vi "Measurement Logic.vi"() -> ()   [LabVIEW 2022 SP3, in "Efficiency Sweep_Class D Amplifier.lvlib"]
uses:
  Efficiency Sweep_Class D Amplifier.lvlib
  Measurement Results.ctl
  <vilib>/Analysis/NI_AALBase.lvlib
  <instrlib>/niDCPower/nidcpower.llb/niDCPower Source Mode.ctl
  <instrlib>/niDCPower/nidcpower.llb/niDCPower Output Function.ctl
  <instrlib>/niDMM/nidmm.llb/niDMM Function.ctl
  <instrlib>/niDMM/nidmm.llb/niDMM Resolution in Digits.ctl
  <vilib>/Analysis/1siggen.llb/Ramp Pattern by Samples.vi
  <instrlib>/niDMM/nidmm.llb/niDMM Configure Measurement Digits.vi
  <vilib>/Plug-In SDKs/Measurements/Measure Call Context/Measure Call Context.lvclass
  Measurement Configuration.ctl
  shared/controls/weighting filter.ctl
  shared/controls/lowpass filter.ctl
  shared/controls/highpass filter.ctl
  shared/controls/units - snr.ctl
  shared/controls/audio controls.lvlib
  shared/controls/units - ratio.ctl
  shared/controls/digital output level units.ctl
  shared/controls/power measurement method.ctl
panel:
  out "XY Graph":cluster{"Array":dbl[], "Array":dbl[]}(graph)
  out "Spectrum":cluster{"x0":dbl, "dx":dbl, "magnitude":dbl[]}[](graph)
  out "Waveform Graph":waveform(dbl)[](graph)
  out "measure call context out":refnum<class "Measure Call Context.lvclass">
  in  "measure call context in":refnum<class "Measure Call Context.lvclass">
  out "measurement results":T1={"channel name"="0", "power supply voltage (V)"=[], "power supply current (A)"=[], "input power (W)"=[], "total output power (W)"=[], "power loss (W)"=[], "efficiency (%)"=[], "wfm - t0"=0.0, "wfm - dt"=1.9531249997269942e-05, "wfm - data"=array[12800 elements], "fft - f0"=0.0, "fft - df"=4.000000000559116, "fft - data"=array[6400 elements]}
  in  "measurement configuration":T2={"digital serial cfg file"="", "digital channel list"="7821\\PCMo 8", "master clock channel list"="7821\\PCMo 0", "output level start"=10.0, "output level stop"=60.0, "output sweep number of steps"=5, "output level units"=enum."% FS", "output range (pk-pk)"=15.0, "load impedance"=4.0, "signal phase"=0.0, "acq sampling rate"=51200.0, "min measurement cycles"=20, "min measurement time (s)"=0.1, "min settling cycles"=0, "min settling time (s)"=0.005, "acq channel"="PXI1Slot4/ai0", "band start"=20.0, "band stop"=20000.0, "weighting filter"=enum."Linear", "highpass filter"=enum."DC", "lowpass filter"=enum."No filter", "SNR units"=enum."dB", "THD+N units"=enum."dB", "THD units"=enum."dB", "gain units"=enum."dB", "power measurement method"=enum."DMM", "power measurement resource"="PXI1Slot9", "power supply voltage"=14.4, "power supply current limit"=1.2, "sense resistor (Ohms)"=0.01} {"band start" format="%0.2f"; "acq sampling rate" format="%0.2f"; "signal phase" format="%#_6p"}
  out "error out":errorcluster
  in  "error in":errorcluster
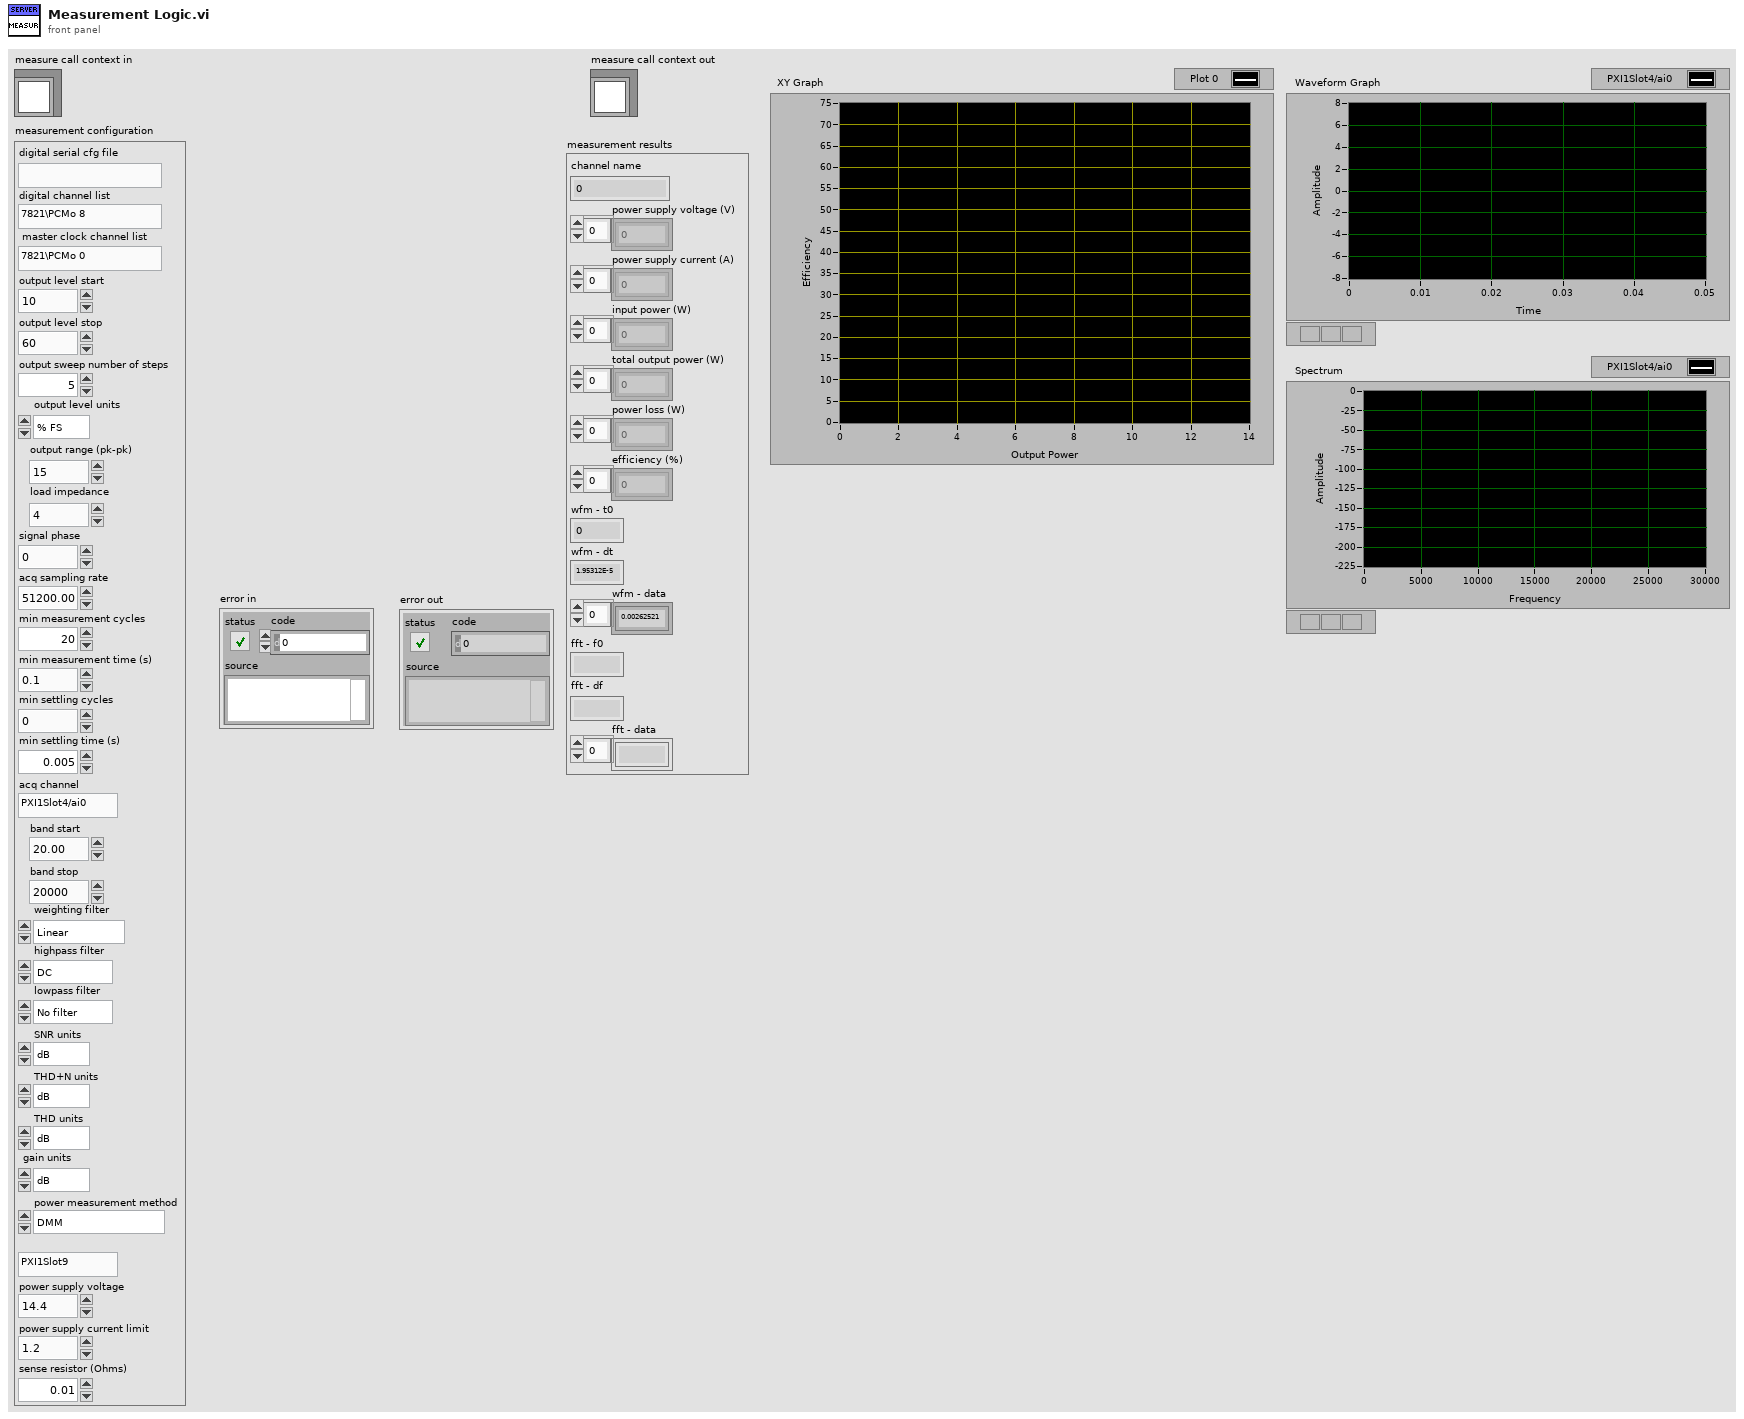
[diagram p1: front panel]
types:
  T1 = typedef "Efficiency Sweep_Class D Amplifier.lvlib/Measurement Results.ctl" = cluster{"channel name":string, "power supply voltage (V)":dbl[], "power supply current (A)":dbl[], "input power (W)":dbl[], "total output power (W)":dbl[], "power loss (W)":dbl[], "efficiency (%)":dbl[], "wfm - t0":dbl, "wfm - dt":dbl, "wfm - data":dbl[], "fft - f0":dbl, "fft - df":dbl, "fft - data":dbl[]}
  T2 = typedef "Efficiency Sweep_Class D Amplifier.lvlib/Measurement Configuration.ctl" = cluster{"digital serial cfg file":string, "digital channel list":string, "master clock channel list":string, "output level start":dbl, "output level stop":dbl, "output sweep number of steps":u32, "output level units":T3, "output range (pk-pk)":dbl, "load impedance":dbl, "signal phase":dbl, "acq sampling rate":dbl, "min measurement cycles":u32, "min measurement time (s)":dbl, "min settling cycles":u32, "min settling time (s)":dbl, "acq channel":string, "band start":dbl, "band stop":dbl, "weighting filter":T4, "highpass filter":T5, "lowpass filter":T6, "SNR units":T7, "THD+N units":T8, "THD units":T8, "gain units":T8, "power measurement method":T9, "power measurement resource":string, "power supply voltage":dbl, "power supply current limit":dbl, "sense resistor (Ohms)":dbl}
  T3 = typedef "audio controls.lvlib/digital output level units.ctl" = enum32{"% FS", "dBFS", "V"}
  T4 = typedef "weighting filter.ctl" = enum32{"Linear", "A-weighting", "B-weighting", "C-weighting"}
  T5 = typedef "highpass filter.ctl" = enum32{"DC", "AC"}
  T6 = typedef "lowpass filter.ctl" = enum32{"No filter", "AES17 20kHz", "AES17 40kHz"}
  T7 = typedef "audio controls.lvlib/units - snr.ctl" = enum32{"dB", "x/y"}
  T8 = typedef "audio controls.lvlib/units - ratio.ctl" = enum32{"dB", "%", "x/y"}
  T9 = typedef "power measurement method.ctl" = enum32{"SMU", "DMM"}
  T10 = typedef "niDMM Function.ctl" = enum16{"DC Volts", "AC Volts", "DC Current", "AC Current", "2-wire Resistance", "4-wire Resistance", "Diode", "Frequency", "Period", "AC Volts DC Coupled", "Capacitance", "Inductance", "Temperature"}
  T11 = typedef "niDCPower Output Function.ctl" = i32
  T12 = typedef "niDCPower Source Mode.ctl" = i32
  T13 = typedef "niDMM Resolution in Digits.ctl" = dbl
  T14 = typedef "single tone measurement settings (HW).ctl" = cluster{"digital channel list":string, "frame clock rate":dbl, "number of channels":u32, "channel length":u32, "bit depth":u32, "data justification":T15, "endianness":T16, "bit clock edge sync":T17, "frame sync edge for channel 0":T17, "channel 0 offset":u32, "master clock channel list":string, "master clock rate":dbl, "enable dither":bool, "logic level":T18, "signal frequency":dbl, "output level":dbl, "output level units":T3, "output range (pk-pk)":dbl, "load impedance":dbl, "signal phase":dbl, "acq sampling rate":dbl, "min measurement cycles":u32, "min measurement time (s)":dbl, "min settling cycles":u32, "min settling time (s)":dbl, "acq channel":string, "band start":dbl, "band stop":dbl, "weighting filter":T4, "highpass filter":T5, "lowpass filter":T6, "SNR units":T7, "THD+N units":T8, "THD units":T8, "gain units":T8}
  T15 = typedef "data justification.ctl" = enum32{"Left Justified", "Right Justified"}
  T16 = typedef "endianness.ctl" = enum32{"MSB First", "LSB First"}
  T17 = typedef "digital edge.ctl" = enum32{"Rising", "Falling"}
  T18 = typedef "logic level.ctl" = enum32{"3.3 V", "1.8 V", "1.2 V"}
  T19 = typedef "PCM tasks.ctl" = cluster{"PCM output task":T20, "PCM output task-clock":T20}
  T20 = typedef "PDM Acquisition Class Library.lvlib/PCM Output Task.lvclass/PCM Output Task DVR.ctl" = refnum<data-value>
  T21 = typedef "audio controls.lvlib/single tone audio measurements.ctl" = cluster{"channel":string, "frequency (Hz)":dbl, "amplitude (Vrms)":dbl, "amplitude (dBFS)":dbl, "phase (deg)":dbl, "SNR":dbl, "THD+N":dbl, "THD":dbl, "dynamic range (dB)":dbl, "gain":dbl, "SFDR (dBc)":dbl}
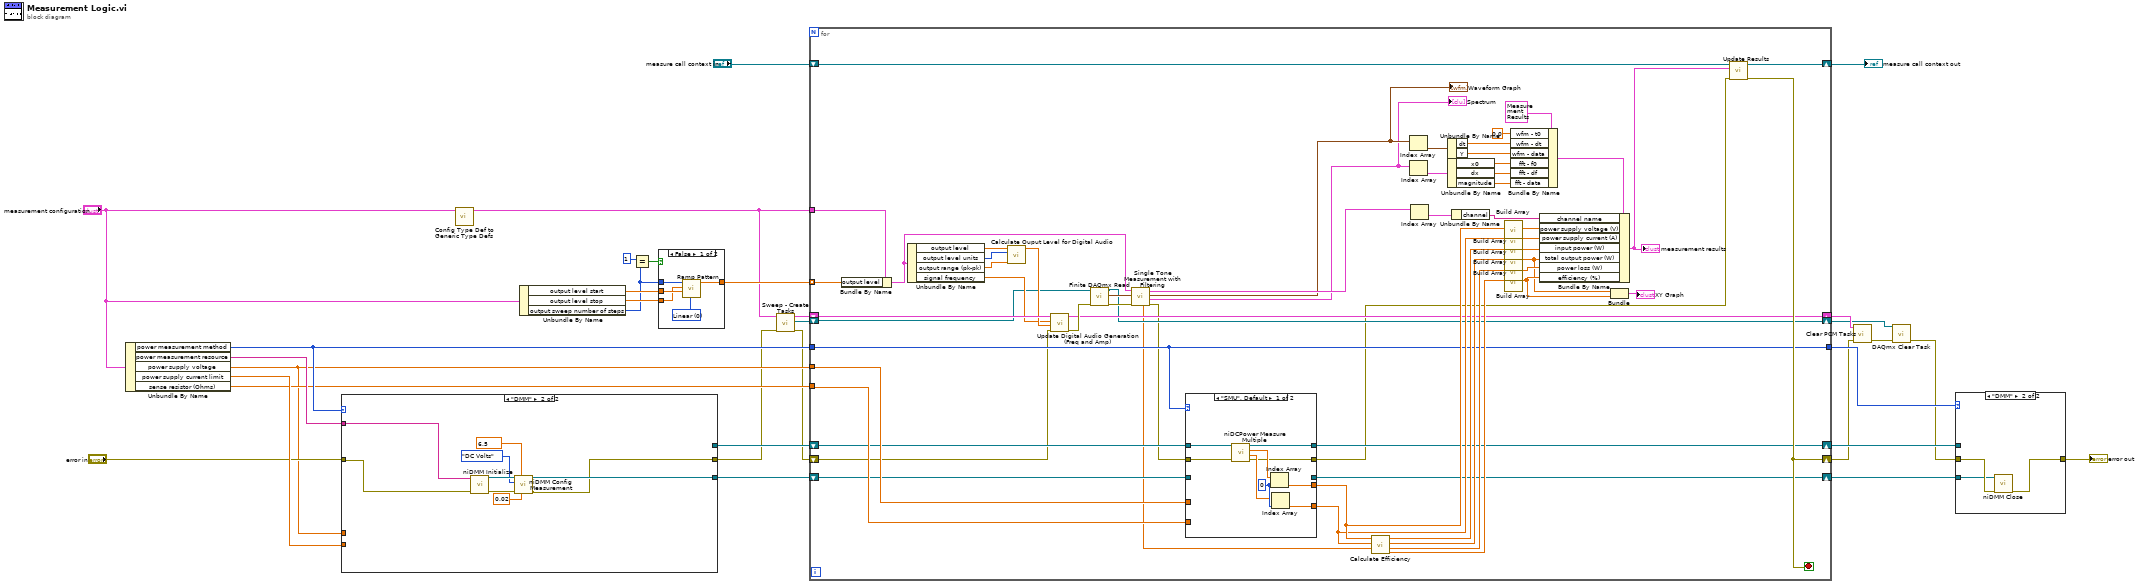
[diagram p0: block diagram]
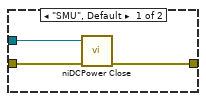
[diagram p2: hidden frame]
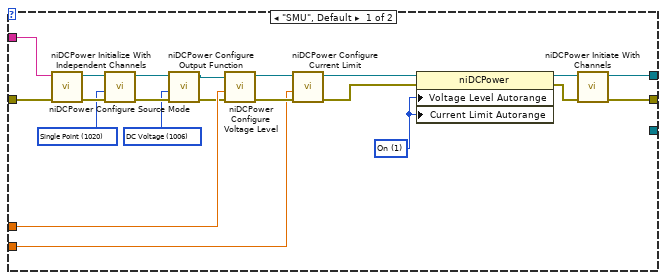
[diagram p3: hidden frame]
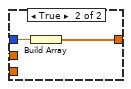
[diagram p4: hidden frame]
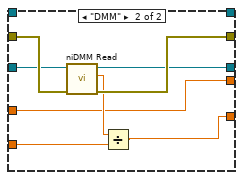
[diagram p5: hidden frame]
diagram:
  n1 = Unbundle By Name("measurement configuration") -> ("power measurement method"=w20:T9, "power measurement resource"=w23:string, "power supply voltage"=w18:dbl, "power supply current limit"=w22:dbl, "sense resistor (Ohms)"=w19:dbl)
  n2 = case shown="\"DMM\"" w20 {
    tunnel: w18 -> [w50 _]
    tunnel: w22 -> [w49 _]
    tunnel: [w35 _] -> w11
    tunnel: [w34 w57] -> w10
    tunnel: "error in" -> [w33 w61]
    tunnel: [_ w58] -> w12
    tunnel: w23 -> [w32 w53]
    frame "SMU", Default {
      w36 = 1 items=["Off", "On"] ("Source:DC Voltage:Current Limit Autorange")
      w37 = T11 1006 items=["DC Voltage"=1006, "DC Current"=1007, "Pulse Voltage"=1049, "Pulse Current"=1050] ("output function")
      w44 = T12 1020 items=["Single Point"=1020, "Sequence"=1021] ("source mode")
      n3 = call <instrlib>:"niDCPower Initialize With Independent Channels.vi"("error in (no error)"=w33, "resource name"=w32) -> ("error out"=w48:errorcluster, "instrument handle out"=w47:refnum<k15>)  [unwired: 8 in]
      n4 = call <instrlib>:"niDCPower Configure Source Mode.vi"("error in (no error)"=w48, "source mode"=w44, "instrument handle"=w47) -> ("error out"=w46:errorcluster, "instrument handle out"=w45:refnum<k15>)  [unwired: 7 out]
      n5 = call <instrlib>:"niDCPower Configure Output Function.vi"("error in (no error)"=w46, "output function"=w37, "instrument handle"=w45) -> ("error out"=w38:errorcluster, "instrument handle out"=w39:refnum<k15>)  [unwired: 1 in, 6 out]
      n6 = call <instrlib>:"niDCPower Configure Voltage Level.vi"("error in (no error)"=w38, "voltage level"=w50, "instrument handle"=w39) -> ("error out"=w51:errorcluster, "instrument handle out"=w52:refnum<k15>)  [unwired: 1 in, 6 out]
      n7 = call <instrlib>:"niDCPower Configure Current Limit.vi"("error in (no error)"=w51, "current limit"=w49, "instrument handle"=w52) -> ("error out"=w40:errorcluster, "instrument handle out"=w43:refnum<k15>)  [unwired: 2 in, 5 out]
      n8 = property class="niDCPower"(reference=w43, error in=w40, "Voltage Level Autorange"=w36, "Current Limit Autorange"=w36) -> (reference out=w42:refnum<k15>, error out=w41:errorcluster)
      n9 = call <instrlib>:"niDCPower Initiate With Channels.vi"("error in (no error)"=w41, "instrument handle"=w42) -> ("error out"=w34:errorcluster, "instrument handle out"=w35:refnum<k15>)  [unwired: 8 in]
    }
    frame "DMM" {
      w55 = T13 6.5 items=["3 1/2"=3.5, "4 1/2"=4.5, "5 1/2"=5.5, "6 1/2"=6.5, "7 1/2"=7.5] ("Resolution in Digits")
      n10 = call <instrlib>:"niDMM Initialize.vi"("error in (no error)"=w61, "Instrument Descriptor"=w53) -> ("error out"=w60:errorcluster, "instrument handle out"=w59:refnum<k15>)  [unwired: 8 in]
      n11 = call-poly <instrlib>:"niDMM Config Measurement.vi"("Range"=0.02, "Resolution in Digits"=w55, "error in (no error)"=w60, "Function"=niDMM_Function."DC Volts", "instrument handle"=w59) -> ("error out"=w57:errorcluster, "instrument handle out"=w58:refnum<k15>)  [unwired: 5 in]
    }
  }
  n12 = call "Config Type Def to Generic Type Defs.vi"("measurement configuration"="measurement configuration") -> ("single tone settings"=w9:T14)  [unwired: 9 in, 1 out]
  n13 = Unbundle By Name("measurement configuration") -> ("output level start"=w31:dbl, "output level stop"=w30:dbl, "output sweep number of steps"=w26:u32)
  n14 = Equal?(x=u32 1, y=w26) -> (x = y?=w27:bool)
  n15 = case shown="False" w27 {
    tunnel: w31 -> [w66 w68]
    tunnel: w30 -> [w65 _]
    tunnel: w26 -> [w64 _]
    tunnel: [w63 w67] -> w29
    frame False {
      w62 = u16 0 items=["Linear", "Logarithmic"] ("type")
      n16 = call-poly <vilib>:"Ramp Pattern.vi"("type"=w62, "start"=w66, "end"=w65, "samples"=w64) -> ("Ramp Pattern"=w63:dbl[])  [unwired: 6 in, 1 out]
    }
    frame True {
      n17 = Build Array(w68) -> (w67:dbl[])
    }
  }
  n18 = call "Sweep - Create Tasks.vi"("error in (no error)"=w10, "measurement configuration"=w9) -> ("error out"=w6:errorcluster, "DAQmx task"=w7:refnum<k21>, "PCM tasks"=w8:T19)  [unwired: 7 in]
  n19 = for {
    tunnel: w29 -> [w98] mode=indexing
    shift-right: [w97] -> w2
    shift-left: w6 -> [w73]
    shift-right: [w126] -> w28
    shift-left: "measure call context in" -> [w125]
    tunnel: w20 -> [w96]
    tunnel: w19 -> [w115]
    tunnel: w18 -> [w114]
    tunnel: w9 -> [w99]
    tunnel: [w96] -> w15
    shift-right: [w95] -> w14
    shift-left: w11 -> [w89]
    shift-right: [w94] -> w13
    shift-left: w12 -> [w90]
    shift-right: [w81] -> w4
    shift-left: w8 -> [w82]
    shift-right: [w77] -> w3
    shift-left: w7 -> [w76]
    stop <- w97 stop-if-true
    n20 = Bundle By Name(cluster=w99, "output level"=w98) -> (w78:T14)
    n21 = Unbundle By Name(w78) -> ("output level"=w88:dbl, "output level units"=w87:T3, "output range (pk-pk)"=w86:dbl, "signal frequency"=w79:dbl)
    n22 = call "Calculate Ouput Level for Digital Audio.vi"("output range (pk-pk)"=w86, "digital output level units"=w87, "output level"=w88) -> ("gain"=w80:dbl)  [unwired: 7 in, 1 out]
    n23 = call "Update Digital Audio Generation (Freq and Amp).vi"("error in (no error)"=w73, "gain"=w80, "frequency"=w79, "PCM tasks"=w82) -> ("error out"=w85:errorcluster, "PCM tasks"=w81:T19)  [unwired: 6 in]
    n24 = call "Finite DAQmx Read.vi"("error in (no error)"=w85, "task/channels in"=w76) -> ("error out"=w84:errorcluster, "data"=w83:waveform(dbl)[], "task out"=w77:refnum<k21>)  [unwired: 7 in]
    n25 = call "Single Tone Measurement with Filtering.vi"("error in (no error)"=w84, "waveforms"=w83, "measurement configuration"=w78) -> ("error out"=w75:errorcluster, "spectra"=w69:cluster{"x0":dbl, "dx":dbl, "magnitude":dbl[]}[], "waveforms"=w70:waveform(dbl)[], "results"=w71:T21[], "output power"=w72:dbl[])  [unwired: 4 in]
    "Waveform Graph" <- w70
    "Spectrum" <- w69
    n26 = case shown="\"SMU\", Default" w96 {
      tunnel: [w135 _] -> w95
      tunnel: [w134 w136] -> w109
      tunnel: [w133 w140] -> w108
      tunnel: [w129 w142] -> w74
      tunnel: w75 -> [w128 w143]
      tunnel: [_ w139] -> w94
      tunnel: w90 -> [_ w138]
      tunnel: w89 -> [w127 _]
      tunnel: w115 -> [_ w137]
      tunnel: w114 -> [_ w136]
      frame "SMU", Default {
        w132 = 0 ("index")
        n27 = call <instrlib>:"niDCPower Measure Multiple.vi"("error in (no error)"=w128, "instrument handle"=w127) -> ("error out"=w129:errorcluster, "current measurements"=w130:dbl[], "voltage measurements"=w131:dbl[], "instrument handle out"=w135:refnum<k15>)  [unwired: 6 in]
        n28 = Index Array(array=w131, index=w132) -> (element=w134:dbl)
        n29 = Index Array(array=w130, index=w132) -> (element=w133:dbl)
      }
      frame "DMM" {
        n30 = call <instrlib>:"niDMM Read.vi"("error in (no error)"=w143, "instrument handle"=w138) -> ("error out"=w142:errorcluster, "Measurement"=w141:dbl, "instrument handle out"=w139:refnum<k15>)  [unwired: 7 in]
        n31 = Divide(x=w141, y=w137) -> (x/y=w140:dbl)
      }
    }
    n32 = call "Calculate Efficiency.vi"("output power per channel"=w72, "power supply current"=w108, "power supply voltage"=w109) -> ("efficiency"=w104:dbl, "power loss"=w105:dbl, "total output power"=w106:dbl, "input power"=w107:dbl)  [unwired: 5 in]
    n33 = Index Array(array=w70) -> (element=w103:waveform(dbl))  [unwired: 1 in]
    n34 = Index Array(array=w69) -> (element=w102:cluster{"x0":dbl, "dx":dbl, "magnitude":dbl[]})  [unwired: 1 in]
    n35 = Index Array(array=w71) -> (element=w101:T21)  [unwired: 1 in]
    n36 = Unbundle By Name(w103) -> ("dt"=w120:dbl, "Y"=w119:dbl[])
    n37 = Unbundle By Name(w102) -> ("x0"=w118:dbl, "dx"=w117:dbl, "magnitude"=w116:dbl[])
    n38 = Unbundle By Name(w101) -> ("channel"=w100:string)
    n39 = call "Build Array.vi"("value"=w109) -> ("Array"=w113:dbl[])  [unwired: 10 in]
    n40 = call "Build Array.vi"("value"=w108) -> ("Array"=w112:dbl[])  [unwired: 10 in]
    n41 = call "Build Array.vi"("value"=w107) -> ("Array"=w111:dbl[])  [unwired: 10 in]
    n42 = call "Build Array.vi"("value"=w106) -> ("Array"=w92:dbl[])  [unwired: 10 in]
    n43 = call "Build Array.vi"("value"=w105) -> ("Array"=w110:dbl[])  [unwired: 10 in]
    n44 = call "Build Array.vi"("value"=w104) -> ("Array"=w93:dbl[])  [unwired: 10 in]
    n45 = Bundle By Name(cluster=T1 {"channel name"="", "power supply voltage (V)"=[], "power supply current (A)"=[], "input power (W)"=[], "total output power (W)"=[], "power loss (W)"=[], "efficiency (%)"=[], "wfm - t0"=0.0, "wfm - dt"=0.0, "wfm - data"=[], "fft - f0"=0.0, "fft - df"=0.0, "fft - data"=[]} ("Measurement Results"), "wfm - t0"=0.0, "wfm - dt"=w120, "wfm - data"=w119, "fft - f0"=w118, "fft - df"=w117, "fft - data"=w116) -> (w122:T1)
    n46 = Bundle By Name(cluster=w122, "channel name"=w100, "power supply voltage (V)"=w113, "power supply current (A)"=w112, "input power (W)"=w111, "total output power (W)"=w92, "power loss (W)"=w110, "efficiency (%)"=w93) -> (w121:T1)
    "measurement results" <- w121
    n47 = Bundle("Array"=w92, "Array"=w93) -> (→"XY Graph":cluster{"Array":dbl[], "Array":dbl[]})  [unwired: 1 in]
    n48 = call <vilib>:"Update Results.vi"("error in"=w74, "measurement results"=w121, "measure call context in"=w125) -> ("error out"=w97:errorcluster, "measure call context out"=w126:refnum<class "Measure Call Context.lvclass">)  [unwired: 7 in]
  }
  "measure call context out" <- w28
  n49 = call "Clear PCM Tasks.vi"("error in (no error)"=w2, "PCM tasks"=w4) -> ("error out"=w5:errorcluster)  [unwired: 9 in]
  n50 = call <vilib>:"DAQmx Clear Task.vi"("task in"=w3, "error in"=w5) -> ("error out"=w1:errorcluster)  [unwired: 13 in]
  n51 = case shown="\"DMM\"" w15 {
    tunnel: [w146 w148] -> w16
    tunnel: w1 -> [w145 w149]
    tunnel: w14 -> [w144 _]
    tunnel: w13 -> [_ w147]
    frame "SMU", Default {
      n52 = call <instrlib>:"niDCPower Close.vi"("error in (no error)"=w145, "instrument handle"=w144) -> ("error out"=w146:errorcluster)  [unwired: 9 out]
    }
    frame "DMM" {
      n53 = call <instrlib>:"niDMM Close.vi"("error in (no error)"=w149, "instrument handle"=w147) -> ("error out"=w148:errorcluster)  [unwired: 9 in]
    }
  }
  "error out" <- w16
